vi "_Blacken.vi"(11 "DialogClose":refnum<user-event>) -> ()   [LabVIEW 2012, in "Dialog.lvlib" / "Dialog.lvclass"]
doc: "This VI is used to create a blackened background around the dialog box."
uses:
  Dialog.lvclass
  Fading/SetTransparency(U8).vi
  Fading/_Fade(I32).vi
panel:
  in  "Transparency (40)":u8=40
types:
  T1 = enum32{"Invalid", "Standard", "Closed", "Hidden", "Minimized", "Maximized"}
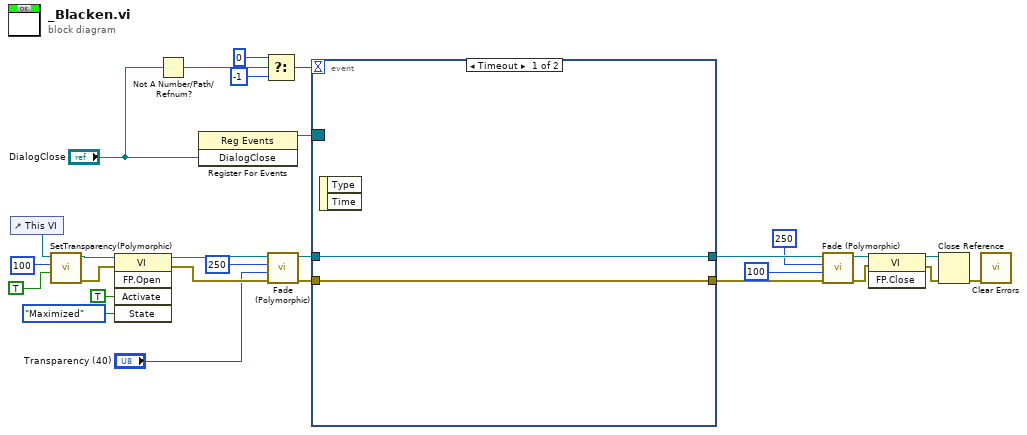
[diagram p0: block diagram]
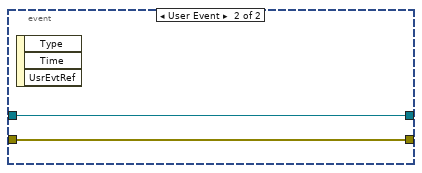
[diagram p2: hidden frame]
diagram:
  n1 = control-ref of="This VI"() -> (w9:refnum<vi>)
  n2 = call-poly "SetTransparency(Polymorphic).vi"("Run VI Transparently (T)"=TRUE, "Transparency (%)"=u8 100, "VI Reference (calling VI)"=w9) -> ("error out"=w23:errorcluster, "dup VI Reference"=w10:refnum<vi>)  [unwired: 1 in, 6 out]
  n3 = invoke class="VI" method="FP.Open"(reference=w10, error in=w23, "Activate"=TRUE ("Activate?"), "State"=T1."Maximized") -> (reference out=w21:refnum<vi>, error out=w20:errorcluster)  [unwired: 1 in, 3 out]
  n4 = Not A Number/Path/Refnum?(number/path/refnum="DialogClose") -> (NaN/Path/Refnum?=w4:bool)
  n5 = register-events("DialogClose") -> (reference out=w26:refnum<event-registration>)  [unwired: 2 in, 1 out]
  n6 = Select(t=0 ("Timeout (-1)"), s=w4, f=-1 ("Timeout (-1)")) -> (s? t:f=w8:i32)
  n7 = call-poly "Fade (Polymorphic).vi"("error in"=w20, "Target Transparency (0)"="Transparency (40)", "Fade time (ms)"=250, "VI Reference (calling VI)"=w21) -> ("error out"=w19:errorcluster, "dup VI Reference"=w18:refnum<vi>)  [unwired: 1 in, 5 out]
  n8 = event shown="[0] Timeout" {
    selector: w26 -> [_ _]
    dyn-events: _ -> [_ _]
    timeout: w8 -> [_ _]
    tunnel: w18 -> [w30 w32]
    tunnel: [w30 w32] -> w17
    tunnel: w19 -> [w29 w31]
    tunnel: [w29 w31] -> w14
    event Timeout {
      n9 = event-data() -> ()  [unwired: 3 out]
    }
    event User Event {
      n10 = event-data() -> ()  [unwired: 4 out]
    }
  }
  n11 = call-poly "Fade (Polymorphic).vi"("error in"=w14, "Target Transparency (0)"=u8 100, "Fade time (ms)"=250, "VI Reference (calling VI)"=w17) -> ("error out"=w13:errorcluster, "dup VI Reference"=w12:refnum<vi>)  [unwired: 1 in, 5 out]
  n12 = invoke class="VI" method="FP.Close"(reference=w12, error in=w13) -> (reference out=w3:refnum<vi>, error out=w2:errorcluster)  [unwired: 1 in, 1 out]
  n13 = Close Reference(reference=w3, error in (no error)=w2) -> (error out=w1:errorcluster)
  n14 = call <vilib>:"Clear Errors.vi"("error in (no error)"=w1) -> ()  [unwired: 7 out]
